vi "RFH-utility-split_data.vi"(7 "Frequency":dbl=1000000000.0, 11 "Common Format":T1) -> (2 "After":T1, 3 "Before":T1)   [LabVIEW 2020, in "RFH-Reflection_File_Handler.lvlib"]
doc: "Splits a Common Format cluster at a frequency into the data before and after it."
uses:
  RFH-Reflection_File_Handler.lvlib
  RFH-common_data_format.ctl
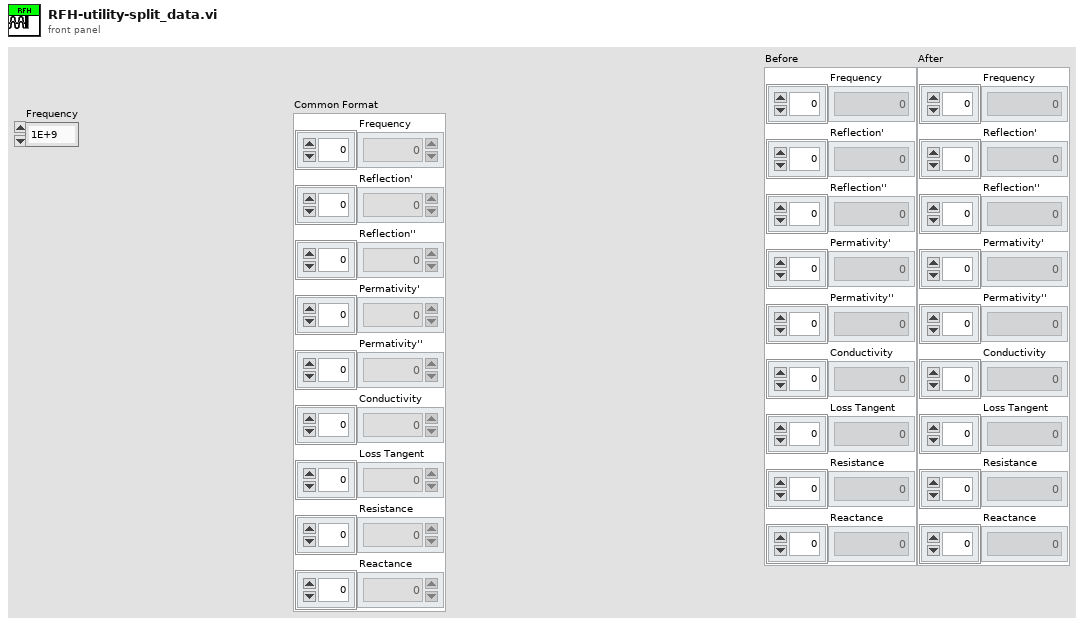
[diagram p1: front panel]
types:
  T1 = typedef "RFH-Reflection_File_Handler.lvlib/RFH-common_data_format.ctl" = cluster{"Frequency":dbl[], "Reflection'":dbl[], "Reflection''":dbl[], "Permativity'":dbl[], "Permativity''":dbl[], "Conductivity":dbl[], "Loss Tangent":dbl[], "Resistance":dbl[], "Reactance":dbl[]}
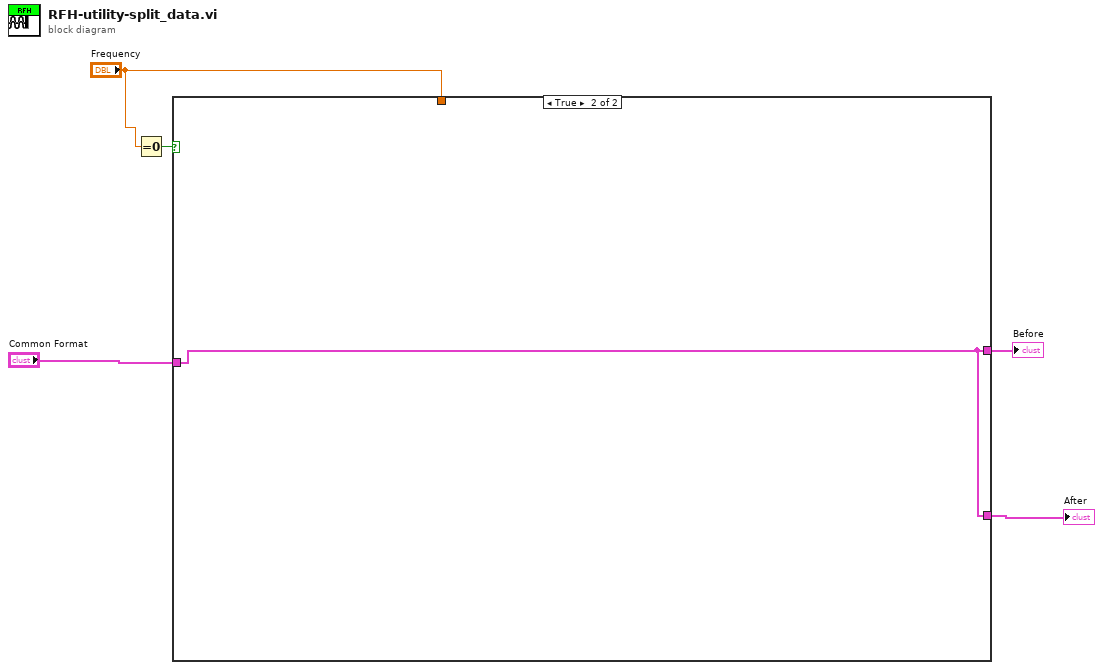
[diagram p0: block diagram]
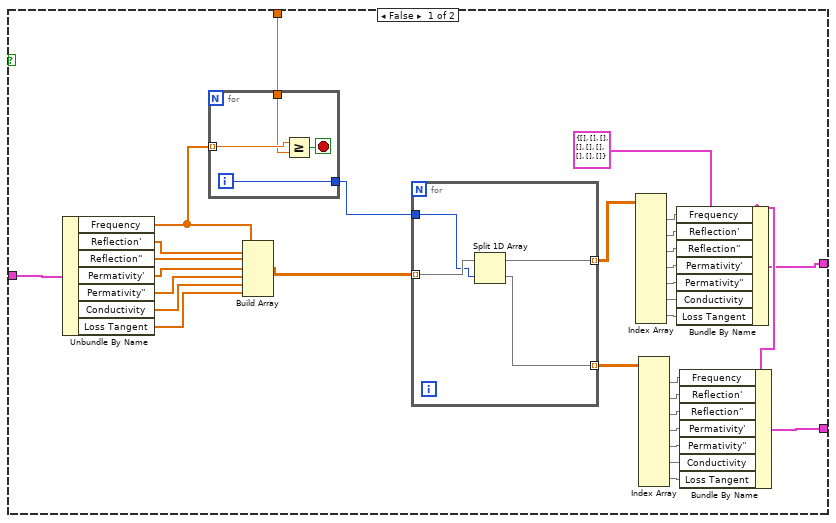
[diagram p2: hidden frame]
diagram:
  n1 = Equal To 0?(x="Frequency") -> (x = 0?=w1:bool)
  n2 = case shown="True" w1 {
    tunnel: "Common Format" -> [w35 w44]
    tunnel: "Frequency" -> [w27 _]
    tunnel: [w7 w44] -> w4
    tunnel: [w6 w44] -> w3
    frame False {
      w8 = T1 {"Frequency"=[], "Reflection'"=[], "Reflection''"=[], "Permativity'"=[], "Permativity''"=[], "Conductivity"=[], "Loss Tangent"=[], "Resistance"=[], "Reactance"=[]} ("Common Format")
      n3 = Unbundle By Name(w35) -> ("Frequency"=w28:dbl[], "Reflection'"=w34:dbl[], "Reflection''"=w33:dbl[], "Permativity'"=w32:dbl[], "Permativity''"=w31:dbl[], "Conductivity"=w30:dbl[], "Loss Tangent"=w29:dbl[])
      n4 = for {
        tunnel: w28 -> [w43] mode=indexing
        tunnel: w27 -> [w42]
        tunnel: [w40] -> w26
        i -> [w40]
        stop <- w41 stop-if-true
        n5 = Greater Or Equal?(x=w43, y=w42) -> (x >= y?=w41:bool)
      }
      n6 = Build Array(w28, w34, w33, w32, w31, w30, w29) -> (w25:dbl[][])
      n7 = for {
        tunnel: w26 -> [w38]
        tunnel: w25 -> [w39] mode=indexing
        tunnel: [w37] -> w24 mode=indexing
        tunnel: [w36] -> w9 mode=indexing
        n8 = Split 1D Array(array=w39, index=w38) -> (first subarray=w37:dbl[], second subarray=w36:dbl[])
      }
      n9 = Index Array(array=w24) -> (element #1=w23:dbl[], element #2=w22:dbl[], element #3=w21:dbl[], element #4=w20:dbl[], element #5=w19:dbl[], element #6=w18:dbl[], element #7=w17:dbl[])  [unwired: 14 in]
      n10 = Index Array(array=w9) -> (element #1=w10:dbl[], element #2=w11:dbl[], element #3=w12:dbl[], element #4=w13:dbl[], element #5=w14:dbl[], element #6=w15:dbl[], element #7=w16:dbl[])  [unwired: 14 in]
      n11 = Bundle By Name(cluster=w8, "Frequency"=w23, "Reflection'"=w22, "Reflection''"=w21, "Permativity'"=w20, "Permativity''"=w19, "Conductivity"=w18, "Loss Tangent"=w17) -> (w7:T1)
      n12 = Bundle By Name(cluster=w8, "Frequency"=w10, "Reflection'"=w11, "Reflection''"=w12, "Permativity'"=w13, "Permativity''"=w14, "Conductivity"=w15, "Loss Tangent"=w16) -> (w6:T1)
    }
    frame True {
    }
  }
  "Before" <- w4
  "After" <- w3
